vi "Environment Variable for PPL venv--constant.vi"(8 "error in":errorcluster) -> (0 "error out":errorcluster, 3 "Environment Variable for Main venv":string="py2vi_tool_venv")   [LabVIEW 2026]
doc: "This constant describes the environment variable that defines the path to the virtual environment that is used by an arbitrary ppl."
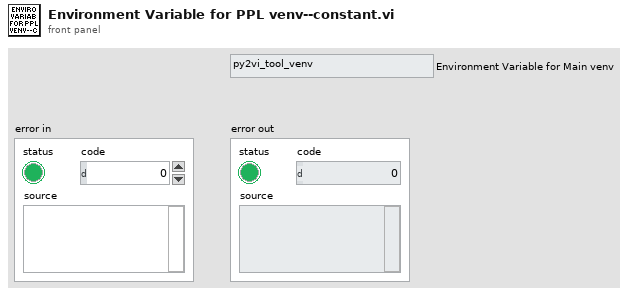
[diagram p1: front panel]
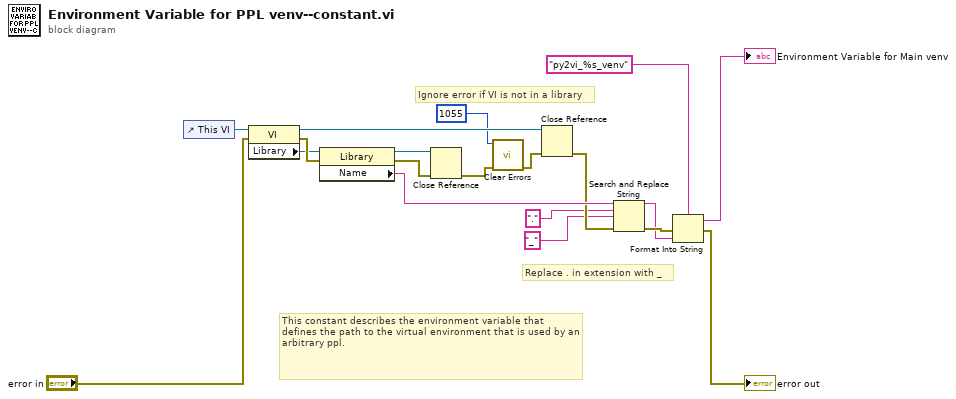
[diagram p0: block diagram]
diagram:
  # "Replace . in extension with _"
  # "Ignore error if VI is not in a library"
  # "This constant describes the environment variable that defines the path to the virtual environment that is used by an arbitrary ppl."
  n1 = control-ref of="This VI"() -> (w13:refnum<vi>)
  n2 = property class="VI"(reference=w13, error in="error in") -> (reference out=w10:refnum<vi>, error out=w19:errorcluster, "Library"=w12:refnum<vi>)
  n3 = property class="Library"(reference=w12, error in=w19) -> (reference out=w11:refnum<vi>, error out=w16:errorcluster, "Name"=w6:string)
  n4 = Close Reference(reference=w11, error in (no error)=w16) -> (error out=w15:errorcluster)
  n5 = call <vilib>:"Clear Errors.vi"("error in (no error)"=w15, "specific error code to clear (0: all)"=1055) -> ("error out"=w14:errorcluster)  [unwired: 4 in, 1 out]
  n6 = Close Reference(reference=w10, error in (no error)=w14) -> (error out=w5:errorcluster)
  n7 = Search and Replace String(input string=w6, search string=".", replace string="_" ("replace string (\"\")"), error in=w5) -> (result string=w3:string, error out=w4:errorcluster)  [unwired: 4 in, 2 out]
  n8 = Format Into String(format string="py2vi_%s_venv", error in=w4, w3) -> (resulting string=→"Environment Variable for Main venv":string, error out=→"error out":errorcluster)  [unwired: 1 in]
